vi "SMTP Email Send Multiple Attachments.vi"(0 "recipients":string[](array[string]) caption="destinataires", 1 "mail server":string caption="serveur mail", 2 "return address":string caption="adresse de retour", 5 "subject ([No Subject])":string="[Sans objet]" caption="objet ([Sans objet])", 7 "message":string, 9 "attachments":T1(array[cluster]) caption="pièces jointes", 11 "error in (no error)":errorcluster caption="entrée d'erreur (pas d'erreur)") -> (4 "invalid recipients":string[](array[string]) caption="destinataires non valides", 15 "error out":errorcluster caption="sortie d'erreur")   [LabVIEW 2022 SP3, in "Copie de NI_SMTPEmail.lvlib"]
doc: "LabVIEW ne supporte plus ce VI. À la place, utilisez le VI Express Envoyer un e-mail.\n\nEnvoie un e-mail avec plusieurs fichiers et des données en pièce jointe à une liste de destinataires.\n\n<b>adresse de retour</b> est l'adresse-email de l'expéditeur du message. Si vous ne spécifiez pas d'adresse de retour, une chaîne vide est envoyée au serveur. Vous n'êtes pas obligé d'inclure une adresse de retour pour que ce VI fonctionne, mais certains serveurs de messagerie n'acceptent pas les messages si ces informations sont absentes. \n<b>serveur mail</b> est le nom ou l'adresse IP d'un serveur SMTP valide. Si vous passez une chaîne vide à cette entrée, LabVIEW n'accepte pas la connexion réseau et renvoie l'erreur 63. \n<b>destinataires</b> est le tableau de chaînes qui contient les adresses e-mail des destinataires du message. Chaque adresse peut être un élément de tableau séparé. \n<b>objet</b> est la ligne d'objet du message. La valeur par défaut est [Sans objet]. \n<b>message</b> correspond au message textuel de l'e-mail, formaté avec le jeu de caractères système. LabVIEW convertit cette chaîne en format UTF-8 avant d'envoyer l'e-mail. \n<b>pièces jointes</b> spécifie le type, l'emplacement et le contenu des pièces jointes à l'e-mail. \n\n<b>chemin</b> spécifie le chemin du fichier que vous voulez mettre en pièce jointe. Entrez Pas un chemin si vous voulez attacher des données plutôt qu'un fichier. \n<b>données</b> contient les données que vous voulez attacher si vous définissez <b>chemin</b> à Pas un chemin. \n<b>binaire</b>, quand il est VRAI (valeur par défaut), indique à LabVIEW d'envoyer les pièces jointes dans le mode binaire. \n<b>type de contenu MIME</b> détermine le type de contenu pour une pièce jointe de type binaire au message. Vous pouvez spécifier n'importe quel type de contenu supporté par la norme RFC 2045, y compris les types de contenu courants suivants :\n\napplication/octet-stream (valeur par défaut) : indique un fichier binaire générique.\n\nimage/jpeg : indique des images JPEG.\n\ntext/html : indique des documents au format HTML.\n\n<b>entrée d'erreur</b> contient les informations sur l'erreur. Cette entrée fournit la fonctionnalité d'entrée d'erreur standard. \n<b>destinataires non valides</b> liste les destinataires rejetés par le serveur mail. \n<b>sortie d'erreur</b> contient des informations sur l'erreur. Cette sortie fournit la fonctionnalité de sortie d'erreur standard."
uses:
  Copie de NI_SMTPEmail.lvlib
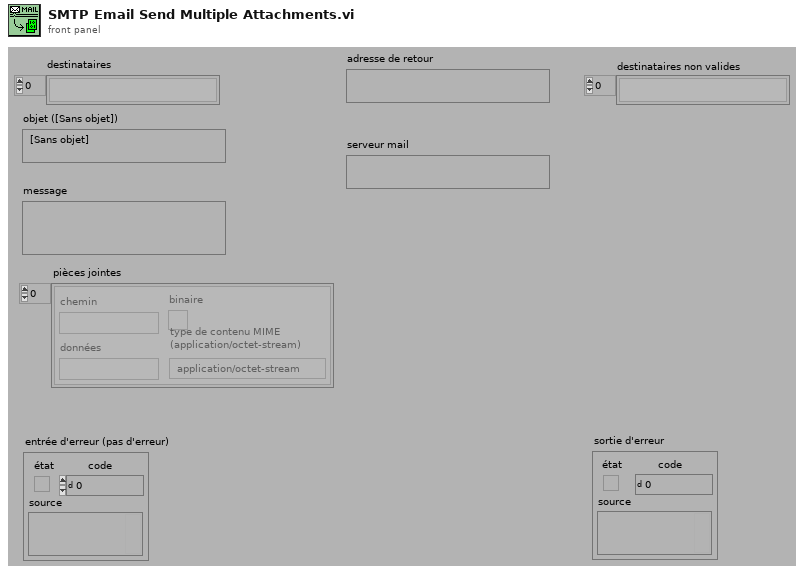
[diagram p1: front panel]
types:
  T1 = cluster{"path":path, "data":string, "binary":bool, "MIME content-type \n(application/octet-stream)":string}[]
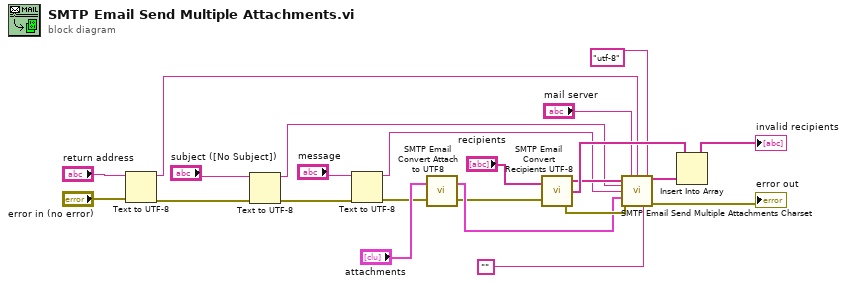
[diagram p0: block diagram]
diagram:
  n1 = Text to UTF-8(8:"error in (no error)", 11:"return address") -> (0:w19:errorcluster, 3:w10:string)  [unwired: 1 in]
  n2 = Text to UTF-8(8:w19, 11:"subject ([No Subject])") -> (0:w21:errorcluster, 3:w8:string)  [unwired: 1 in]
  n3 = Text to UTF-8(8:w21, 11:"message") -> (0:w3:errorcluster, 3:w7:string)  [unwired: 1 in]
  n4 = call "SMTP Email Convert Attach to UTF8.vi"("error in"=w3, "attachments"="attachments") -> ("error out"=w2:errorcluster, "UTF-8 Attachments"=w4:T1)
  n5 = call "SMTP Email Convert Recipients UTF-8.vi"("recipients"="recipients", "error in"=w2) -> ("convertible recipients"=w12:string[], "unconvertible recipients"=w13:string[], "error out"=w16:errorcluster)
  n6 = call "SMTP Email Send Multiple Attachments Charset.vi"("recipients"=w12, "mail server"="mail server", "return address"=w10, "character set (us-ascii)"="utf-8", "subject ([No Subject])"=w8, "message"=w7, "attachments"=w4, "error in (no error)"=w16, "translit"="") -> ("invalid recipients"=w17:string[], "error out"=→"error out":errorcluster)  [unwired: 5 in]
  n7 = Insert Into Array(array=w13, new element=w17) -> (→"invalid recipients":string[])  [unwired: 1 in]
